vi "When Method One Return Value.vi"(0 "error out":errorcluster, 2 "Return Value":dbl, 8 "error in (no error)":errorcluster, 11 "Test Interface Mock In":refnum<class "Test Interface Mock.lvclass">) -> (3 "Test Interface Mock Out":refnum<class "Test Interface Mock.lvclass">)   [LabVIEW 2020, in "Test Interface Mock.lvclass"]
uses:
  Test Interface Mock.lvclass
  C:/git/astemes-lmock/source/Framework/Mock/LMock Mock.lvclass
  source/Framework/Mock/LMock Mock.lvclass
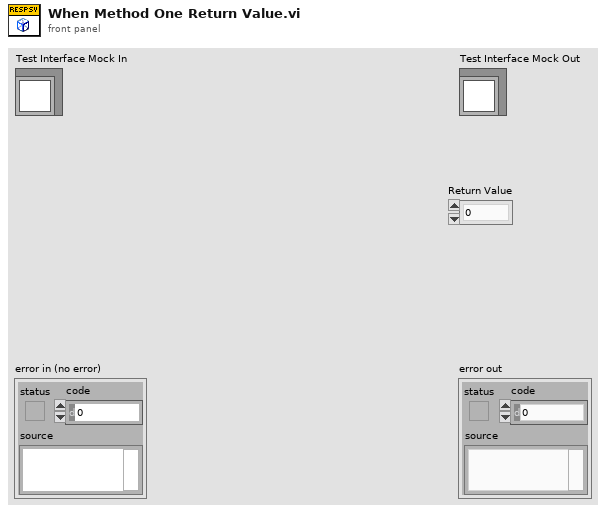
[diagram p1: front panel]
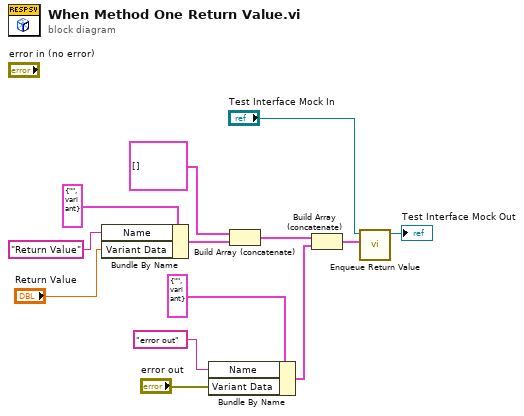
[diagram p0: block diagram]
diagram:
  n1 = Bundle By Name(cluster=cluster{"Name":string, "Variant Data":variant} {"Name"="", "Variant Data"=variant} ("element"), "Name"="Return Value", "Variant Data"="Return Value") -> (w3:cluster{"Name":string, "Variant Data":variant})
  n2 = Bundle By Name(cluster=cluster{"Name":string, "Variant Data":variant} {"Name"="", "Variant Data"=variant} ("element"), "Name"="error out", "Variant Data"="error out") -> (w1:cluster{"Name":string, "Variant Data":variant})
  n3 = Build Array (concatenate)(cluster{"Name":string, "Variant Data":variant}[] [] ("Control Values"), w3) -> (w9:cluster{"Name":string, "Variant Data":variant}[])
  n4 = Build Array (concatenate)(w9, w1) -> (w8:cluster{"Name":string, "Variant Data":variant}[])
  n5 = call "Enqueue Return Value.vi"("Indicator Values"=w8, "Mock In"="Test Interface Mock In") -> ("Mock Out"=→"Test Interface Mock Out":refnum<class "Test Interface Mock.lvclass">)  [unwired: 8 in, 1 out]
